vi "Replace Outside Typedef Control.vi"(6 "dependent vis":path[](array[path]), 8 "error in":errorcluster, 9 "shared directory":path, 10 "non-library vi[]":string[](array[string]), 11 "measurement directory":path) -> (0 "error out":errorcluster)   [LabVIEW 2021, in "Multiple Converter.lvlib"]
uses:
  Multiple Converter.lvlib
  Converter Reusables/Converter Reusables.lvlib
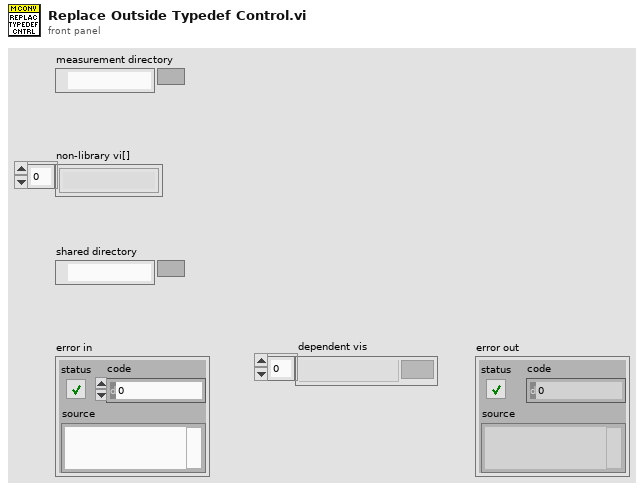
[diagram p1: front panel]
types:
  T1 = enum32{"not a typedef", "typedef", "strict typedef", "class private data"}
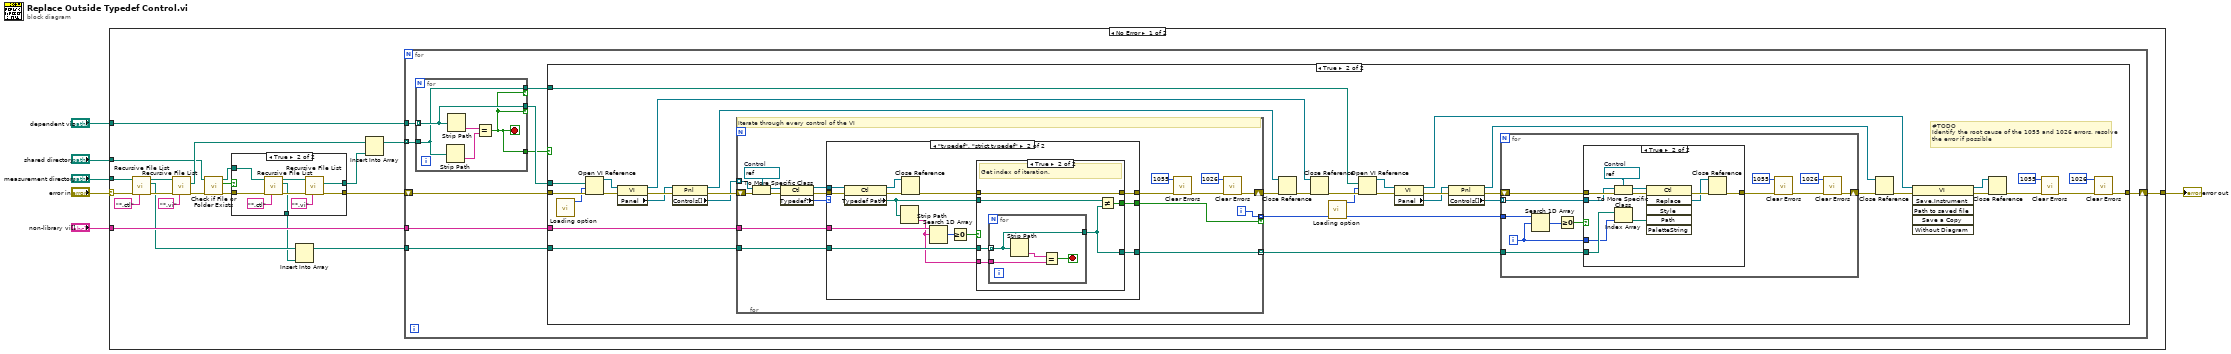
[diagram p0: block diagram]
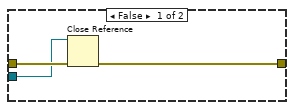
[diagram p3: hidden frame]
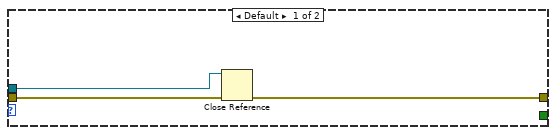
[diagram p4: hidden frame]
diagram:
  n1 = case shown="No Error" "error in" {
    selector: "error in" -> [w26 w162]
    tunnel: "non-library vi[]" -> [w27 _]
    tunnel: [w24 w162] -> w4
    tunnel: "measurement directory" -> [w22 _]
    tunnel: "shared directory" -> [w8 _]
    tunnel: "dependent vis" -> [w7 _]
    frame No Error {
      n2 = call <vilib>:"Recursive File List.vi"("pattern"="*.ctl", "error in (no error)"=w26, "Folder Path"=w22) -> ("error out"=w23:errorcluster, "All Files in Dir"=w19:path[], "dup Folder Path"=w21:path)  [unwired: 4 in, 2 out]
      n3 = call <vilib>:"Recursive File List.vi"("pattern"="*.vi", "error in (no error)"=w23, "Folder Path"=w21) -> ("error out"=w17:errorcluster, "All Files in Dir"=w16:path[])  [unwired: 4 in, 3 out]
      n4 = call <vilib>:"Check if File or Folder Exists.vi"("error in (no error)"=w17, "path"=w8) -> ("error out"=w11:errorcluster, "file or folder exists?"=w10:bool, "dup path"=w9:path)  [unwired: 7 in]
      n5 = case shown="True" w10 {
        tunnel: [w152 w157] -> w18
        tunnel: w11 -> [w152 w156]
        tunnel: [_ w155] -> w13
        tunnel: [_ w154] -> w12
        tunnel: w9 -> [_ w153]
        frame False {
        }
        frame True {
          n6 = call <vilib>:"Recursive File List.vi"("pattern"="*.ctl", "error in (no error)"=w156, "Folder Path"=w153) -> ("error out"=w159:errorcluster, "All Files in Dir"=w155:path[], "dup Folder Path"=w160:path)  [unwired: 4 in, 2 out]
          n7 = call <vilib>:"Recursive File List.vi"("pattern"="*.vi", "error in (no error)"=w159, "Folder Path"=w160) -> ("error out"=w157:errorcluster, "All Files in Dir"=w154:path[])  [unwired: 4 in, 3 out]
        }
      }
      n8 = Insert Into Array(array=w19, new element=w13) -> (w14:path[])  [unwired: 1 in]
      n9 = Insert Into Array(array=w16, new element=w12) -> (w15:path[])  [unwired: 1 in]
      n10 = for {
        tunnel: w14 -> [w36]
        tunnel: w27 -> [w35]
        tunnel: w15 -> [w33] mode=indexing
        shift-right: [w29] -> w24
        shift-left: w18 -> [w31]
        tunnel: w7 -> [w34]
        n11 = for {
          tunnel: w34 -> [w149] mode=indexing
          tunnel: w33 -> [w148]
          tunnel: [w149] -> w32 if=w147
          tunnel: [w148] -> w30 if=w147
          tunnel: [w147] -> w28
          stop <- w147 stop-if-true
          n12 = Strip Path(path=w148) -> (name=w150:string)  [unwired: 1 out]
          n13 = Strip Path(path=w149) -> (name=w151:string)  [unwired: 1 out]
          n14 = Equal?(x=w151, y=w150) -> (x = y?=w147:bool)
        }
        n15 = case shown="True" w28 {
          tunnel: w36 -> [_ w74]
          tunnel: w35 -> [_ w73]
          tunnel: w32 -> [_ w69]
          tunnel: w31 -> [w37 w68]
          tunnel: w30 -> [_ w50]
          tunnel: [w37 w60] -> w29
          frame False {
          }
          frame True {
            # "#TODO\nIdentify the root cause of the 1055 and 1026 errors, resolve \nthe error if possible"
            n16 = call "Loading option.vi"() -> ("options"=w39:i32)  [unwired: 11 in]
            n17 = Open VI Reference(vi path=w69, options=w39, error in (no error)=w68) -> (vi reference=w64:refnum<vi>, error out=w65:errorcluster)  [unwired: 3 in]
            n18 = property class="VI"(reference=w64, error in=w65) -> (reference out=w53:refnum<vi>, error out=w66:errorcluster, "Panel"=w63:refnum<vi>)
            n19 = property class="Pnl"(reference=w63, error in=w66) -> (reference out=w54:refnum<vi>, error out=w62:errorcluster, "Controls[]"=w56:refnum<vi>[])
            n20 = for {
              tunnel: w56 -> [w118] mode=indexing
              tunnel: w73 -> [w115]
              tunnel: w74 -> [w117]
              shift-right: [w105] -> w55
              shift-left: w62 -> [w110]
              tunnel: [w103] -> w43 mode=indexing
              tunnel: [w101] -> w44 mode=indexing if=w102
              i -> [w101]
              w116 = refnum<vi> refnum  # Control
              # "Iterate through every control of the VI"
              n21 = To More Specific Class(target class=w116, reference=w118, error in=w110) -> (specific class reference=w114:refnum<vi>, error out=w104:errorcluster)
              n22 = property class="Ctl"(reference=w114, error in=w104) -> (reference out=w112:refnum<vi>, error out=w113:errorcluster, "Typedef?"=w111:T1)
              n23 = case shown="\"typedef\", \"strict typedef\"" w111 {
                tunnel: w113 -> [w121 w125]
                tunnel: w112 -> [w119 w130]
                tunnel: [w120 w134] -> w109
                tunnel: w117 -> [_ w132]
                tunnel: w115 -> [_ w131]
                tunnel: [_ w123] -> w103
                tunnel: [_ w122] -> w102
                frame Default {
                  n24 = Close Reference(reference=w119, error in (no error)=w121) -> (error out=w120:errorcluster)
                }
                frame "typedef", "strict typedef" {
                  n25 = property class="Ctl"(reference=w130, error in=w125) -> (reference out=w126:refnum<vi>, error out=w127:errorcluster, "Typedef Path"=w128:path)
                  n26 = Strip Path(path=w128) -> (name=w129:string)  [unwired: 1 out]
                  n27 = Close Reference(reference=w126, error in (no error)=w127) -> (error out=w124:errorcluster)
                  n28 = Search 1D Array(1D array=w131, element=w129) -> (index of element=w135:i32)  [unwired: 1 in]
                  n29 = Greater Or Equal To 0?(x=w135) -> (x >= 0?=w133:bool)
                  n30 = case shown="True" w133 {
                    tunnel: [w136 w140] -> w134
                    tunnel: w132 -> [_ w142]
                    tunnel: w129 -> [_ w141]
                    tunnel: w128 -> [_ w139]
                    tunnel: w124 -> [w136 w140]
                    tunnel: [_ w138] -> w123
                    tunnel: [_ w137] -> w122
                    frame False {
                      # "Pass"
                    }
                    frame True {
                      # "Get index of iteration."
                      n31 = for {
                        tunnel: w142 -> [w143] mode=indexing
                        tunnel: w141 -> [w145]
                        tunnel: [w143] -> w138
                        stop <- w144 stop-if-true
                        n32 = Strip Path(path=w143) -> (name=w146:string)  [unwired: 1 out]
                        n33 = Equal?(x=w146, y=w145) -> (x = y?=w144:bool)
                      }
                      n34 = Not Equal?(x=w139, y=w138) -> (x != y?=w137:bool)
                    }
                  }
                }
              }
              n35 = call <vilib>:"Clear Errors.vi"("error in (no error)"=w109, "specific error code to clear (0: all)"=1055) -> ("error out"=w108:errorcluster)  [unwired: 4 in, 1 out]
              n36 = call <vilib>:"Clear Errors.vi"("error in (no error)"=w108, "specific error code to clear (0: all)"=1026) -> ("error out"=w105:errorcluster)  [unwired: 4 in, 1 out]
            }
            n37 = Close Reference(reference=w54, error in (no error)=w55) -> (error out=w52:errorcluster)
            n38 = Close Reference(reference=w53, error in (no error)=w52) -> (error out=w67:errorcluster)
            n39 = call "Loading option.vi"() -> ("options"=w38:i32)  [unwired: 11 in]
            n40 = Open VI Reference(vi path=w50, options=w38, error in (no error)=w67) -> (vi reference=w48:refnum<vi>, error out=w51:errorcluster)  [unwired: 3 in]
            n41 = property class="VI"(reference=w48, error in=w51) -> (reference out=w40:refnum<vi>, error out=w49:errorcluster, "Panel"=w46:refnum<vi>)
            n42 = property class="Pnl"(reference=w46, error in=w49) -> (reference out=w41:refnum<vi>, error out=w47:errorcluster, "Controls[]"=w45:refnum<vi>[])
            n43 = for {
              tunnel: w45 -> [w82] mode=indexing
              shift-right: [w78] -> w61
              shift-left: w47 -> [w86]
              tunnel: w44 -> [w84]
              tunnel: w43 -> [w81]
              i -> [w75]
              n44 = Search 1D Array(1D array=w84, element=w75) -> (index of element=w80:i32)  [unwired: 1 in]
              n45 = Greater Or Equal To 0?(x=w80) -> (x >= 0?=w83:bool)
              n46 = case shown="True" w83 {
                tunnel: w86 -> [w89 w100]
                tunnel: [w88 w95] -> w85
                tunnel: w82 -> [w87 w93]
                tunnel: w81 -> [_ w92]
                tunnel: w75 -> [_ w90]
                frame False {
                  n47 = Close Reference(reference=w87, error in (no error)=w89) -> (error out=w88:errorcluster)
                }
                frame True {
                  w98 = refnum<vi> refnum  # Control
                  n48 = To More Specific Class(target class=w98, reference=w93, error in=w100) -> (specific class reference=w96:refnum<vi>, error out=w99:errorcluster)
                  n49 = Index Array(array=w92, index=w90) -> (element=w91:path)
                  n50 = invoke class="Ctl" method="Replace"(reference=w96, error in=w99, "Path"=w91) -> (error out=w97:errorcluster, "Replace"=w94:refnum<vi>)  [unwired: 3 in, 4 out]
                  n51 = Close Reference(reference=w94, error in (no error)=w97) -> (error out=w95:errorcluster)
                }
              }
              n52 = call <vilib>:"Clear Errors.vi"("error in (no error)"=w85, "specific error code to clear (0: all)"=1055) -> ("error out"=w79:errorcluster)  [unwired: 4 in, 1 out]
              n53 = call <vilib>:"Clear Errors.vi"("error in (no error)"=w79, "specific error code to clear (0: all)"=1026) -> ("error out"=w78:errorcluster)  [unwired: 4 in, 1 out]
            }
            n54 = Close Reference(reference=w41, error in (no error)=w61) -> (error out=w42:errorcluster)
            n55 = invoke class="VI" method="Save.Instrument"(reference=w40, error in=w42) -> (reference out=w70:refnum<vi>, error out=w71:errorcluster)  [unwired: 4 in, 4 out]
            n56 = Close Reference(reference=w70, error in (no error)=w71) -> (error out=w72:errorcluster)
            n57 = call <vilib>:"Clear Errors.vi"("error in (no error)"=w72, "specific error code to clear (0: all)"=1055) -> ("error out"=w58:errorcluster)  [unwired: 4 in, 1 out]
            n58 = call <vilib>:"Clear Errors.vi"("error in (no error)"=w58, "specific error code to clear (0: all)"=1026) -> ("error out"=w60:errorcluster)  [unwired: 4 in, 1 out]
          }
        }
      }
    }
    frame Error {
    }
  }
  "error out" <- w4
